vi "Sample.vi"(8 "错误输入（无错误）":errorcluster, 10 "VISA资源名称":refnum<visa-resource-name>) -> (0 "error out":errorcluster, 2 "Data Out":dbl[](array[numeric]) format="%.2f")   [LabVIEW 2026, in "UI-湿度测量.lvlib" / "Acquisition.lvlib"]
uses:
  Acquisition.lvlib
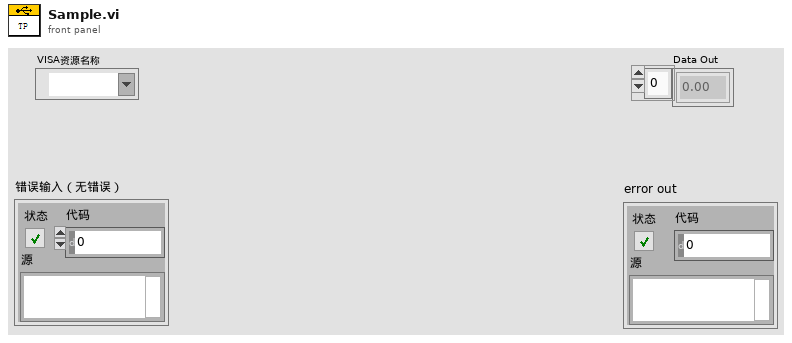
[diagram p1: front panel]
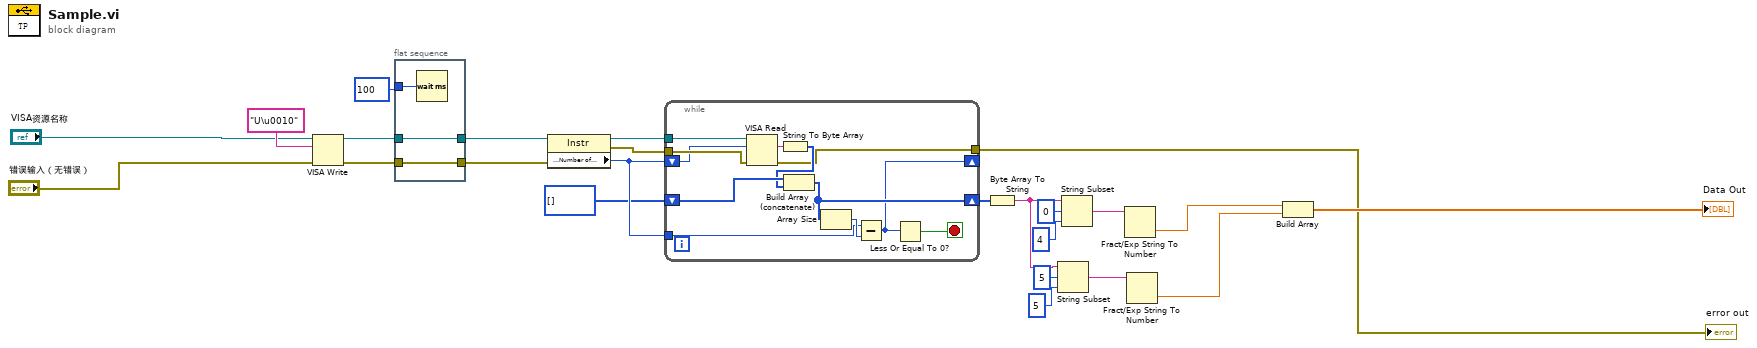
[diagram p0: block diagram]
diagram:
  n1 = VISA Write(VISA resource name="VISA资源名称", write buffer="U\u0010" ("Command"), error in (no error)="错误输入（无错误）") -> (VISA resource name out=w20:refnum<visa-resource-name>, error out=w18:errorcluster)  [unwired: 1 out]
  n2 = flat-sequence {
    tunnel: w18 -> [w26]
    tunnel: [w26] -> w19
    tunnel: w20 -> [w25]
    tunnel: [w25] -> w21
    tunnel: u32 100 ("读取前延时(ms)") -> [w27]
    frame #0 {
      n3 = Wait (ms)(milliseconds to wait=w27) -> ()  [unwired: 1 out]
    }
  }
  n4 = property class="Instr"(reference=w21, error in=w19) -> (reference out=w22:refnum<visa-resource-name>, error out=w23:errorcluster, "Serial Settings:Number of Bytes at Serial Port"=w24:u32)
  n5 = while {
    tunnel: w22 -> [w37]
    tunnel: w23 -> [w36]
    shift-right: [w39] -> w7
    shift-left: u8[] [] ("unsigned byte array") -> [w38]
    tunnel: w24 -> [w31]
    shift-right: [w29] -> _
    shift-left: w24 -> [w35]
    tunnel: [w28] -> w1
    stop <- w30 stop-if-true
    n6 = VISA Read(VISA resource name=w37, byte count=w35, error in (no error)=w36) -> (read buffer=w34:string, error out=w28:errorcluster)  [unwired: 2 out]
    n7 = String To Byte Array(string=w34) -> (unsigned byte array=w33:u8[])
    n8 = Build Array (concatenate)(w38, w33) -> (w39:u8[])
    n9 = Array Size(array=w39) -> (size(s)=w32:i32)
    n10 = Subtract(x=w31, y=w32) -> (x-y=w29:u32)
    n11 = Less Or Equal To 0?(x=w29) -> (x <= 0?=w30:bool)
  }
  "error out" <- w1
  n12 = Byte Array To String(unsigned byte array=w7) -> (string=w10:string)
  n13 = String Subset(string=w10, offset (0)=5 ("偏移量(0)"), length (rest)=5 ("长度（剩余）")) -> (substring=w8:string)
  n14 = String Subset(string=w10, offset (0)=0 ("偏移量(0)"), length (rest)=4 ("长度（剩余）")) -> (substring=w9:string)
  n15 = Fract/Exp String To Number(string=w9) -> (number=w4:dbl)  [unwired: 3 in, 1 out]
  n16 = Fract/Exp String To Number(string=w8) -> (number=w3:dbl)  [unwired: 3 in, 1 out]
  n17 = Build Array(w4, w3) -> (→"Data Out":dbl[])
